vi "Start.vi"(8 "error in (no error)":errorcluster, 10 "Container":refnum<vi>, 11 "ArrayManager in":refnum<class "ArrayManager.lvclass">) -> (0 "error out":errorcluster, 3 "ArrayManager out":refnum<class "ArrayManager.lvclass">)   [LabVIEW 2020, in "OOPanel.lvlib" / "ArrayManager.lvclass"]
uses:
  ArrayManager.lvclass
  ArrayManager.lvclass/ArrayManager.ctl
  Array Panel Async.vi
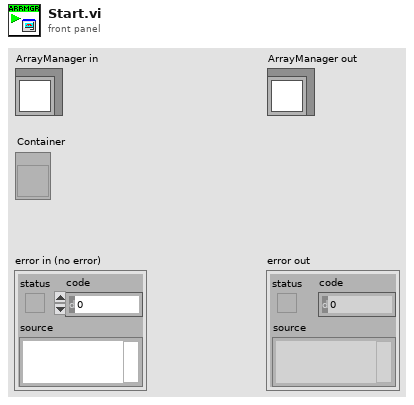
[diagram p1: front panel]
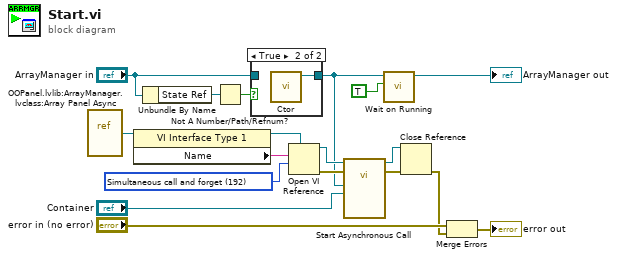
[diagram p0: block diagram]
diagram:
  w12 = 192 items=["Record modifications"=1, "Open templates for editing"=2, "Prompt user to save"=4, "Prepare for reentrant run"=8, "Prompt to find missing subVIs"=16, "Hide loading dialog box"=32, "Enable simultaneous calls"=64, "Prepare to call and forget"=128, "Simultaneous call and forget"=192, "Prepare to call and collect"=256, "Simultaneous call and collect"=320]
  n1 = vi-ref "OOPanel.lvlib:ArrayManager.lvclass:Array Panel Async.vi"() -> (w10:refnum<vi>)
  n2 = property class="VI Interface Type 1"(reference=w10) -> (reference out=w13:refnum<vi>, "Name"=w11:string)  [unwired: 1 in, 1 out]
  n3 = Unbundle By Name("ArrayManager in") -> ("State Ref"=w4:refnum<data-value>)
  n4 = Not A Number/Path/Refnum?(number/path/refnum=w4) -> (NaN/Path/Refnum?=w3:bool)
  n5 = case shown="True" w3 {
    tunnel: "ArrayManager in" -> [w19 _]
    tunnel: [w19 w20] -> w1
    frame False {
    }
    frame True {
      n6 = call "Ctor.vi"() -> ("PanelArray"=w20:refnum<class "ArrayManager.lvclass">)  [unwired: 10 in, 1 out]
    }
  }
  n7 = Open VI Reference(type specifier VI Refnum (for type only)=w13, vi path=w11, options=w12) -> (vi reference=w15:refnum<vi>, error out=w14:errorcluster)  [unwired: 3 in]
  n8 = call-by-ref "Start Asynchronous Call"(reference=w15, error in=w14, "Container"="Container", "PanelArray in"=w1) -> (reference out=w17:refnum<vi>, error out=w16:errorcluster)  [unwired: 10 in]
  n9 = call "Wait on Running.vi"("Value"=TRUE, "ArrayManager in"=w1) -> ("ArrayManager out"=→"ArrayManager out":refnum<class "ArrayManager.lvclass">)  [unwired: 8 in, 1 out]
  n10 = Close Reference(reference=w17, error in (no error)=w16) -> (error out=w5:errorcluster)
  n11 = Merge Errors("error in (no error)", w5) -> (→"error out":errorcluster)
